vi "任意波形脚本.vi"(8 "4-wire":bool, 11 "波形":waveform(dbl)) -> (3 "Script":string)   [LabVIEW 2020, in "功能选择.xctl"]
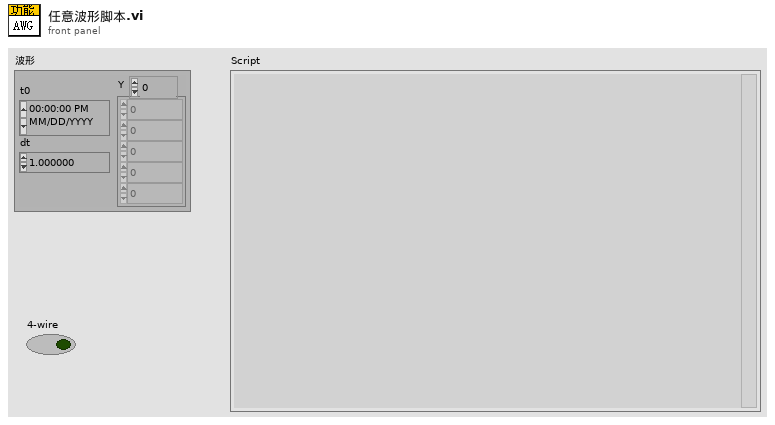
[diagram p1: front panel]
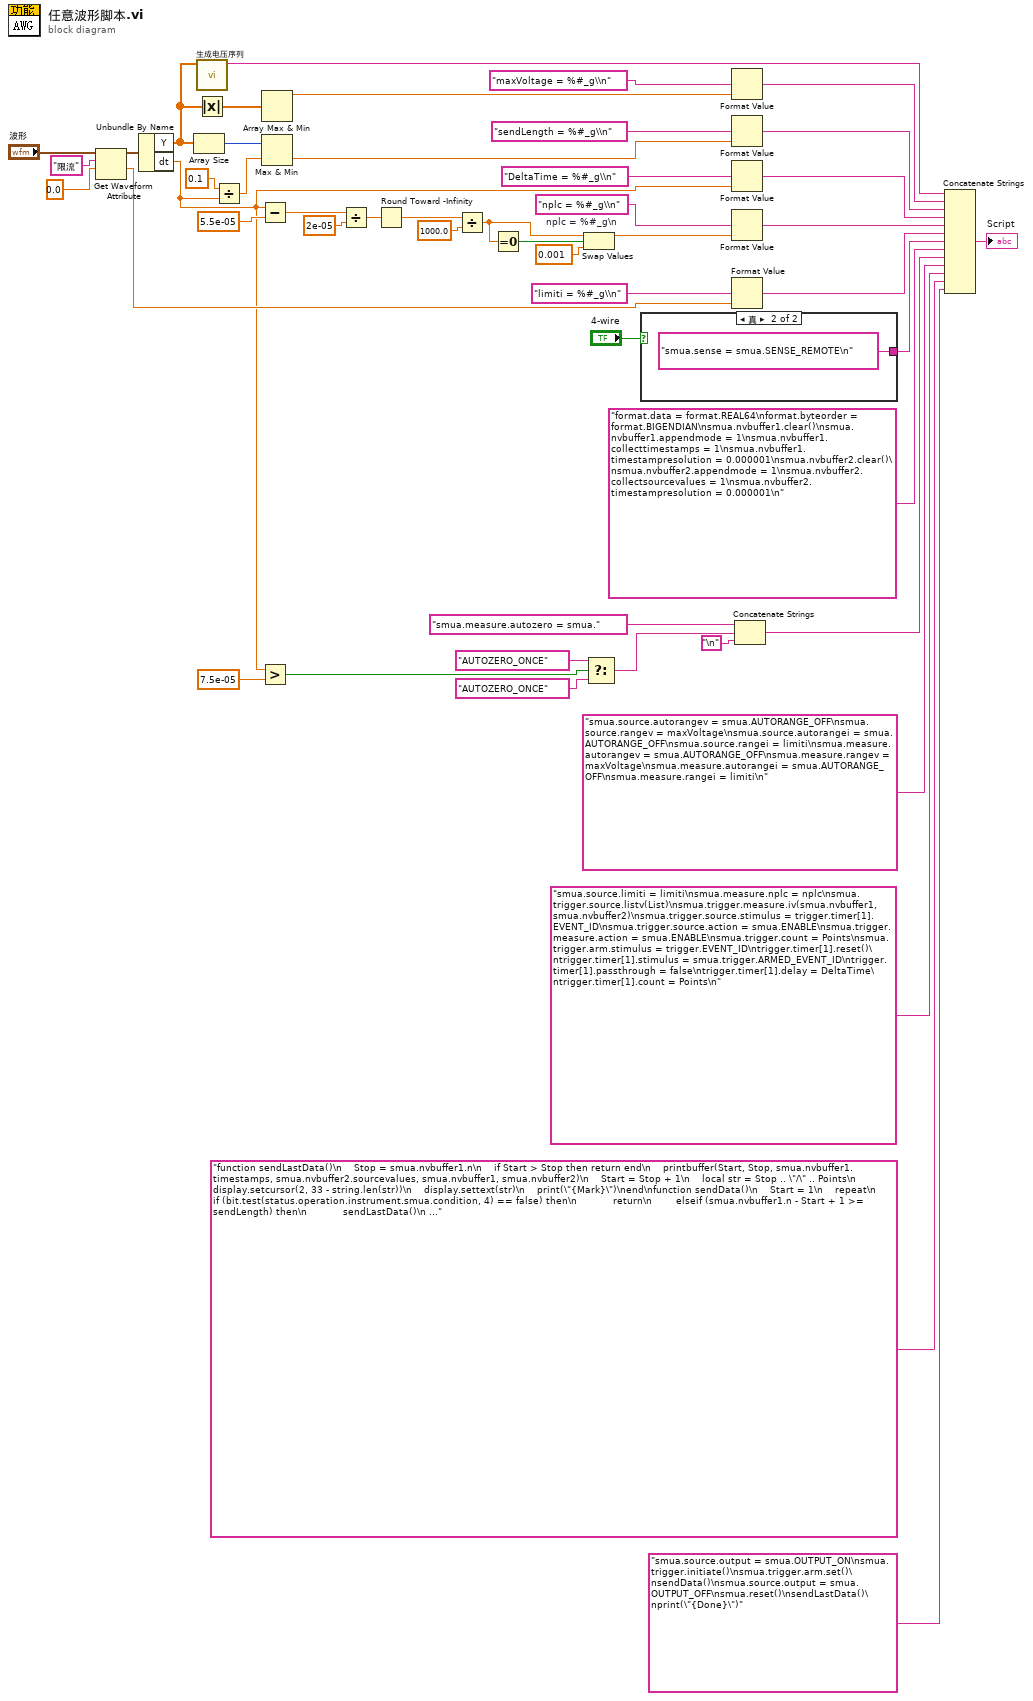
[diagram p0: block diagram]
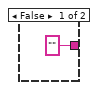
[diagram p2: hidden frame]
diagram:
  w42 = "nplc = %#_g\\n"  # nplc = %#_g\n
  n1 = Get Waveform Attribute(5:0.0, 6:"限流" ("名称"), 7:"波形") -> (1:w22:dbl, 3:w23:waveform(dbl))  [unwired: 1 in, 2 out]
  n2 = Unbundle By Name(w23) -> ("Y"=w33:dbl[], "dt"=w7:dbl)
  n3 = Array Size(array=w33) -> (size(s)=w32:i32)
  n4 = call "生成电压序列.vi"("电压序列"=w33) -> ("List"=w43:string)  [unwired: 10 in]
  n5 = Absolute Value(x=w33) -> (abs(x)=w45:dbl[])
  n6 = Divide(x=0.1, y=w7) -> (x/y=w31:dbl)
  n7 = Subtract(x=w7, y=5.5e-05) -> (x-y=w16:dbl)
  n8 = Greater?(x=w7, y=7.5e-05) -> (0:w5:bool)
  n9 = Array Max & Min(array=w45) -> (max value=w44:dbl)  [unwired: 3 out]
  n10 = Max & Min(x=w32, y=w31) -> (min(x,y)=w30:dbl)  [unwired: 1 out]
  n11 = Divide(x=w16, y=2e-05 ("x")) -> (x/y=w19:dbl)
  n12 = Round Toward -Infinity(1:w19) -> (0:w14:dbl)
  n13 = Divide(x=w14, y=1000.0) -> (x/y=w3:dbl)
  n14 = Equal To 0?(x=w3) -> (x = 0?=w2:bool)
  n15 = Swap Values(12:w3, 13:w2, 14:0.001 ("x/y")) -> (1:w4:dbl)  [unwired: 1 out]
  n16 = Select(t="AUTOZERO_ONCE" ("字符串"), s=w5, f="AUTOZERO_ONCE") -> (s? t:f=w10:string)
  n17 = case shown="真" "4-wire" {
    tunnel: ["" "smua.sense = smua.SENSE_REMOTE\n"] -> w21
    frame False {
    }
    frame True {
    }
  }
  n18 = Format Value(format string="maxVoltage = %#_g\\n" ("格式字符串"), value (0)=w44) -> (output string=w50:string)  [unwired: 1 in]
  n19 = Format Value(format string="sendLength = %#_g\\n" ("格式字符串"), value (0)=w30) -> (output string=w28:string)  [unwired: 1 in]
  n20 = Format Value(format string="DeltaTime = %#_g\\n" ("格式字符串"), value (0)=w7) -> (output string=w48:string)  [unwired: 1 in]
  n21 = Format Value(format string=w42, value (0)=w4) -> (output string=w46:string)  [unwired: 1 in]
  n22 = Format Value(format string="limiti = %#_g\\n" ("格式字符串"), value (0)=w22) -> (output string=w27:string)  [unwired: 1 in]
  n23 = Concatenate Strings("smua.measure.autozero = smua.", w10, "\n") -> (w8:string)
  n24 = Concatenate Strings(w43, w50, w28, w48, w46, w27, w21, "format.data = format.REAL64\nformat.byteorder = format.BIGENDIAN\nsmua.nvbuffer1.clear()\nsmua.nvbuffer1.appendmode = 1\nsmua.nvbuffer1.collecttimestamps = 1\nsmua.nvbuffer1.timestampresolution = 0.000001\nsmua.nvbuffer2.clear()\nsmua.nvbuffer2.appendmode = 1\nsmua.nvbuffer2.collectsourcevalues = 1\nsmua.nvbuffer2.timestampresolution = 0.000001\n", w8, "smua.source.autorangev = smua.AUTORANGE_OFF\nsmua.source.rangev = maxVoltage\nsmua.source.autorangei = smua.AUTORANGE_OFF\nsmua.source.rangei = limiti\nsmua.measure.autorangev = smua.AUTORANGE_OFF\nsmua.measure.rangev = maxVoltage\nsmua.measure.autorangei = smua.AUTORANGE_OFF\nsmua.measure.rangei = limiti\n", "smua.source.limiti = limiti\nsmua.measure.nplc = nplc\nsmua.trigger.source.listv(List)\nsmua.trigger.measure.iv(smua.nvbuffer1, smua.nvbuffer2)\nsmua.trigger.source.stimulus = trigger.timer[1].EVENT_ID\nsmua.trigger.source.action = smua.ENABLE\nsmua.trigger.measure.action = smua.ENABLE\nsmua.trigger.count = Points\nsmua.trigger.arm.stimulus = trigger.EVENT_ID\ntrigger.timer[1].reset()\ntrigger.timer[1].stimulus = smua.trigger.ARMED_EVENT_ID\ntrigger.timer[1].passthrough = false\ntrigger.timer[1].delay = DeltaTime\ntrigger.timer[1].count = Points\n", "function sendLastData()\n    Stop = smua.nvbuffer1.n\n    if Start > Stop then return end\n    printbuffer(Start, Stop, smua.nvbuffer1.timestamps, smua.nvbuffer2.sourcevalues, smua.nvbuffer1, smua.nvbuffer2)\n    Start = Stop + 1\n    local str = Stop .. \"/\" .. Points\n    display.setcursor(2, 33 - string.len(str))\n    display.settext(str)\n    print(\"{Mark}\")\nend\nfunction sendData()\n    Start = 1\n    repeat\n        if (bit.test(status.operation.instrument.smua.condition, 4) == false) then\n            return\n        elseif (smua.nvbuffer1.n - Start + 1 >= sendLength) then\n            sendLastData()\n        end\n        delay(DeltaTime)\n    until (false)\nend\n", "smua.source.output = smua.OUTPUT_ON\nsmua.trigger.initiate()\nsmua.trigger.arm.set()\nsendData()\nsmua.source.output = smua.OUTPUT_OFF\nsmua.reset()\nsendLastData()\nprint(\"{Done}\")") -> (→"Script":string)
